vi "Microscope software version global.vi"() -> ()   [LabVIEW 2015]
panel:
  in  "Version String":string="Version 34  (12/23)"
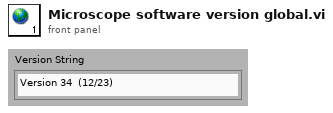
[diagram p1: front panel]
diagram:
